vi "ArmJoystickControl.vi"(0 "Joystick control":T3) -> (1 "TargetPosition":T1, 2 "ArmPlanRequest":T2, 3 "NewPath":bool)   [LabVIEW 2017]
uses:
  TypeDefs/JoystickControls.ctl
  TypeDefs/ArmPlanRequest.ctl
  TypeDefs/ArmTargetPosition.ctl
  ArgosLib/Signal Processing/TypeDefs/EdgeDetector_Type.ctl
  ArgosLib/ArgosLib.lvlib
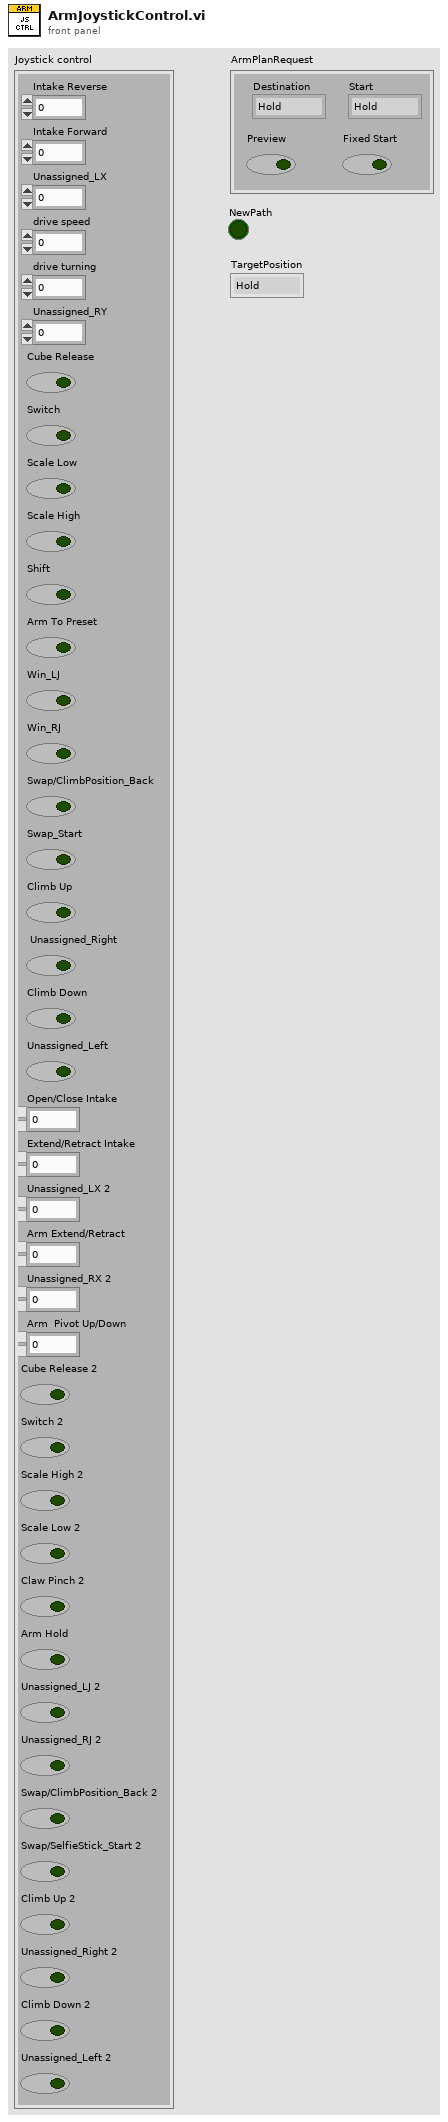
[diagram p1: front panel]
types:
  T1 = typedef "ArmTargetPosition.ctl" = enum16{"Hold", "Switch", "Scale Low", "Scale High", "Climb", "Back Place"}
  T2 = typedef "ArmPlanRequest.ctl" = cluster{"Destination":T1, "Preview":bool, "Start":T1, "Fixed Start":bool}
  T3 = typedef "JoystickControls.ctl" = cluster{"drive speed":dbl, "drive turning":dbl, "Unassigned_LX":dbl, "Unassigned_RY":dbl, "Cube Release":bool, "Intake Forward":dbl, "Intake Reverse ":dbl, "Switch":bool, "Scale Low":bool, "Scale High":bool, "Shift":bool, "Arm To Preset":bool, "Win_LJ":bool, "Win_RJ":bool, "Swap/ClimbPosition_Back":bool, "Swap_Start":bool, "Arm Extend/Retract":dbl, "Unassigned_RX 2":dbl, "Unassigned_LX 2":dbl, "Arm  Pivot Up/Down ":dbl, "Cube Release 2":bool, "Extend/Retract Intake":dbl, "Open/Close Intake":dbl, "Switch 2":bool, "Scale High 2":bool, "Scale Low 2":bool, "Claw Pinch 2":bool, "Arm Hold":bool, "Unassigned_LJ 2":bool, "Unassigned_RJ 2":bool, "Swap/ClimbPosition_Back 2":bool, "Swap/SelfieStick_Start 2":bool, "Climb Up 2":bool, "Unassigned_Right 2":bool, "Climb Down 2":bool, "Unassigned_Left 2":bool, "Climb Up ":bool, " Unassigned_Right":bool, "Climb Down":bool, "Unassigned_Left":bool}
  T4 = typedef "ArgosLib.lvlib/EdgeDetector_Type.ctl" = enum16{"RisingEdge", "FallingEdge", "Both"}
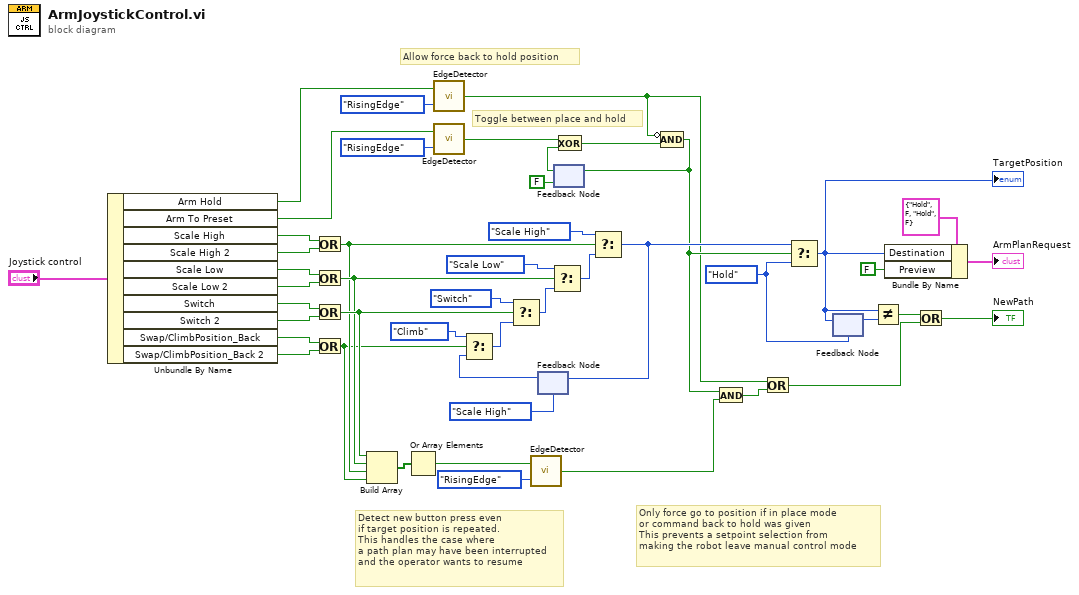
[diagram p0: block diagram]
diagram:
  w25 = ArmTargetPosition."Hold" ("f")
  # "Only force go to position if in place mode\nor command back to hold was given\nThis prevents a setpoint selection from\nmaking the robot leave manual control mode"
  # "Allow force back to hold position"
  # "Detect new button press even\nif target position is repeated.\nThis handles the case where\na path plan may have been interrupted\nand the operator wants to resume"
  # "Toggle between place and hold"
  n1 = Unbundle By Name("Joystick control") -> ("Arm Hold"=w13:bool, "Arm To Preset"=w34:bool, "Scale High"=w46:bool, "Scale High 2"=w45:bool, "Scale Low"=w44:bool, "Scale Low 2"=w43:bool, "Switch"=w42:bool, "Switch 2"=w41:bool, "Swap/ClimbPosition_Back"=w6:bool, "Swap/ClimbPosition_Back 2"=w5:bool)
  n2 = Or(x=w46, y=w45) -> (x .or. y?=w19:bool)
  n3 = Or(x=w44, y=w43) -> (x .or. y?=w20:bool)
  n4 = Or(x=w42, y=w41) -> (x .or. y?=w21:bool)
  n5 = Or(x=w6, y=w5) -> (x .or. y?=w3:bool)
  n6 = Build Array(w21, w20, w19, w3) -> (w18:bool[])
  n7 = Or Array Elements(Boolean array=w18) -> (logical OR=w16:bool)
  n8 = call "EdgeDetector.vi"("DetectorType"=EdgeDetector_Type."RisingEdge", "Input"=w13) -> ("Edge"=w8:bool)
  n9 = call "EdgeDetector.vi"("DetectorType"=EdgeDetector_Type."RisingEdge", "Input"=w34) -> ("Edge"=w30:bool)
  n10 = call "EdgeDetector.vi"("DetectorType"=EdgeDetector_Type."RisingEdge", "Input"=w16) -> ("Edge"=w10:bool)
  n11 = feedback #1(ArmTargetPosition."Scale High" ("ArmTargetPosition")) -> (w2:T1)
  n12 = Select(t=ArmTargetPosition."Climb", s=w3, f=w2) -> (s? t:f=w4:T1)
  n13 = Select(t=ArmTargetPosition."Switch", s=w21, f=w4) -> (s? t:f=w38:T1)
  n14 = Select(t=ArmTargetPosition."Scale Low", s=w20, f=w38) -> (s? t:f=w39:T1)
  n15 = feedback #2(FALSE) -> (w32:bool)
  n16 = Exclusive Or(1:w32, 2:w30) -> (0:w12:bool)
  n17 = Select(t=ArmTargetPosition."Scale High", s=w19, f=w39) -> (s? t:f=w29:T1)
  n18 = feedback-in #1(w29) -> ()
  n19 = Compound Arithmetic op=AND(invert w8, w12) -> (w11:bool)
  n20 = feedback-in #2(w11) -> ()
  n21 = And(x=w11, y=w10) -> (x .and. y?=w9:bool)
  n22 = Or(x=w8, y=w9) -> (x .or. y?=w7:bool)
  n23 = Select(t=w29, s=w11, f=w25) -> (s? t:f=w23:T1)
  "TargetPosition" <- w23
  n24 = feedback-in #3(w23) -> ()
  n25 = feedback #3(w25) -> (w24:T1)
  n26 = Not Equal?(x=w23, y=w24) -> (x != y?=w22:bool)
  n27 = Bundle By Name(cluster=T2 {"Destination"=enum."Hold", "Preview"=FALSE, "Start"=enum."Hold", "Fixed Start"=FALSE} ("ArmPlanRequest"), "Destination"=w23, "Preview"=FALSE) -> (→"ArmPlanRequest":T2)
  n28 = Or(x=w22, y=w7) -> (x .or. y?=→"NewPath":bool)
